vi "XPN Set Calibration Mode.vi"(8 "error in (no error)":errorcluster, 9 "defectMode":i32, 10 "gainMode":i32, 11 "offsetMode":i32) -> (0 "error out":errorcluster, 3 "function return":i32)   [LabVIEW 2022 SP3, in "xPanelWrapper.lvlib"]
doc: "XPN_API int XPN_SetCalibrationMode(int offsetMode, int gainMode, int defectMode);"
uses:
  xPanelWrapper.lvlib
  xPanelWrapper.dll
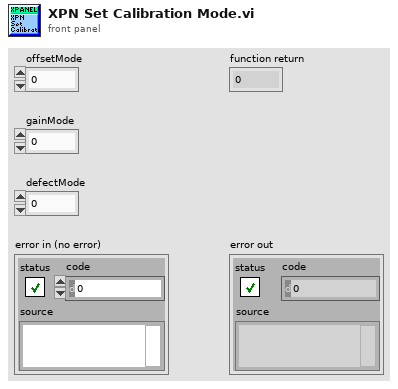
[diagram p1: front panel]
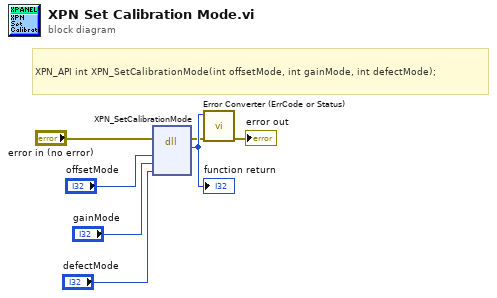
[diagram p0: block diagram]
diagram:
  # "XPN_API int XPN_SetCalibrationMode(int offsetMode, int gainMode, int defectMode);"
  n1 = dll-call lib="E:/SourceCodes/image-harvest/ImageHandler/xPanelWrapperLvLib/xPanelWrapper.*" fn="XPN_SetCalibrationMode"(error in="error in (no error)", "offsetMode"="offsetMode", "gainMode"="gainMode", "defectMode"="defectMode") -> (error out=w2:errorcluster, w7:i32)  [unwired: 5 in, 1 out]
  "function return" <- w7
  n2 = call "Error Converter (ErrCode or Status).vi"("error in (no error)"=w2, "error code"=w7) -> ("error out"=→"error out":errorcluster)  [unwired: 9 in]
